vi "Ch_Merge_Values.vi"(0 "Channels":T1(array[cluster]), 5 "Values":dbl[](array[numeric]), 11 "error in":errorcluster) -> (4 "Channels out":T1(array[cluster]), 15 "error out":errorcluster)   [LabVIEW 2026]
doc: "Values[i]를 Channels[i].Value로 복사(Values가 비면 그대로)."
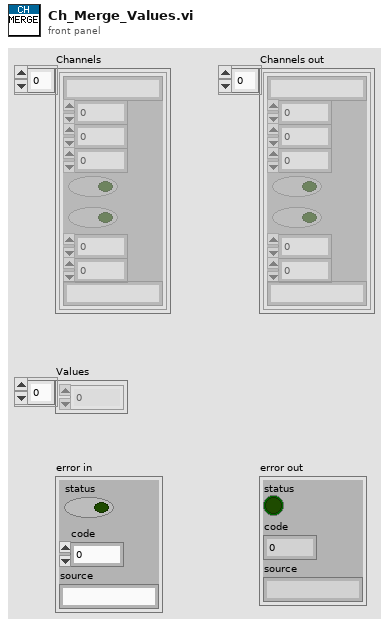
[diagram p1: front panel]
types:
  T1 = cluster{"Name":string, "Value":dbl, "High Limit":dbl, "Low Limit":dbl, "Save":bool, "Graph":bool, "Scale Min":dbl, "Scale Max":dbl, "Unit":string}[]
  T2 = cluster{"Name":string, "Value":dbl, "High Limit":dbl, "Low Limit":dbl, "Save":bool, "Graph":bool, "Scale Min":dbl, "Scale Max":dbl, "Unit":string}
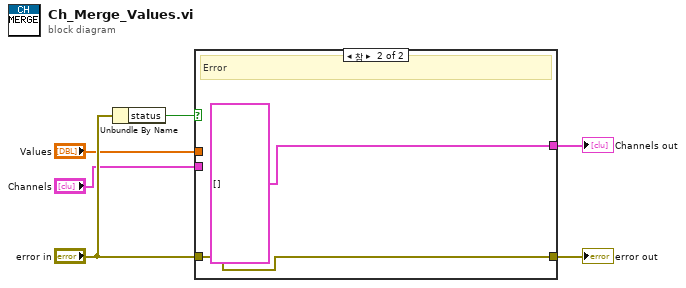
[diagram p0: block diagram]
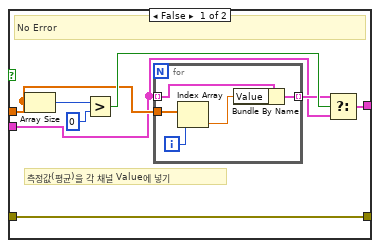
[diagram p2: hidden frame]
diagram:
  n1 = Unbundle By Name("error in") -> ("status"=w4:bool)
  n2 = case shown="참" w4 {
    tunnel: "Channels" -> [w7 _]
    tunnel: "Values" -> [w8 _]
    tunnel: "error in" -> [w9 w20]
    tunnel: [w9 w20] -> w6
    tunnel: [w14 T1 []] -> w5
    frame False {
      # "측정값(평균)을 각 채널 Value에 넣기"
      # "No Error"
      n3 = Array Size(array=w8) -> (size(s)=w11:i32)
      n4 = Greater?(x=w11, y=0) -> (0:w13:bool)
      n5 = for {
        tunnel: w7 -> [w16] mode=indexing
        tunnel: w8 -> [w17]
        tunnel: [w19] -> w10 mode=indexing
        i -> [w15]
        n6 = Index Array(array=w17, index=w15) -> (element=w18:dbl)
        n7 = Bundle By Name(cluster=w16, "Value"=w18) -> (w19:T2)
      }
      n8 = Select(t=w10, s=w13, f=w7) -> (s? t:f=w14:T1)
    }
    frame True {
      # "Error"
    }
  }
  "Channels out" <- w5
  "error out" <- w6
